vi "Build Json.vi"(8 "Error In":errorcluster, 11 "Asset":refnum<class "Asset.lvclass">) -> (0 "Error Out":errorcluster, 2 "JSON File Content":string, 3 "JSON File Name":string)   [LabVIEW 2019, in "Asset.lvclass"]
uses:
  Asset.lvclass
  AssetsJson.ctl
  AssetJson.ctl
  AssetLocationJson.ctl
  AssetExternalCalibrationJson.ctl
  ExternalCalibrationOperatorJson.ctl
  Asset Location/Asset Location.lvclass
  Asset External Calibration/Asset External Calibration.lvclass
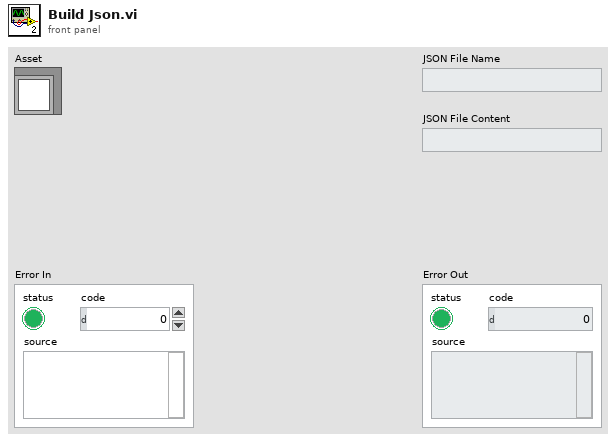
[diagram p1: front panel]
types:
  T1 = typedef "Asset.lvclass/AssetJson.ctl" = cluster{"serialNumber":string, "modelName":string, "modelNumber":u32, "vendorName":string, "vendorNumber":u32, "busType":string, "assetClass":string, "assetName":string, "firmwareVersion":string, "hardwareVersion":string, "location":T2, "supportsExternalCalibration":bool, "externalCalibration":T3, "name":string}
  T2 = typedef "Asset.lvclass/AssetLocationJson.ctl" = cluster{"slotNumber":u32, "parent":string}
  T3 = typedef "Asset.lvclass/AssetExternalCalibrationJson.ctl" = cluster{"date":string, "comments":string, "recommendedInterval":u32, "operator":T4, "temperatureSensors":cluster{"name":string, "reading":dbl}[], "nextRecommendedDate":string}
  T4 = typedef "Asset.lvclass/ExternalCalibrationOperatorJson.ctl" = cluster{"displayName":string, "userId":string}
  T5 = typedef "Asset.lvclass/AssetsJson.ctl" = cluster{"assets":T1[]}
  T6 = typedef "LVDateTimeRec.ctl" = cluster{"fractional second":dbl, "second":i32, "minute":i32, "hour":i32, "day of month":i32, "month":i32, "year":i32, "day of week":i32, "day of year":i32, "DST":i32}
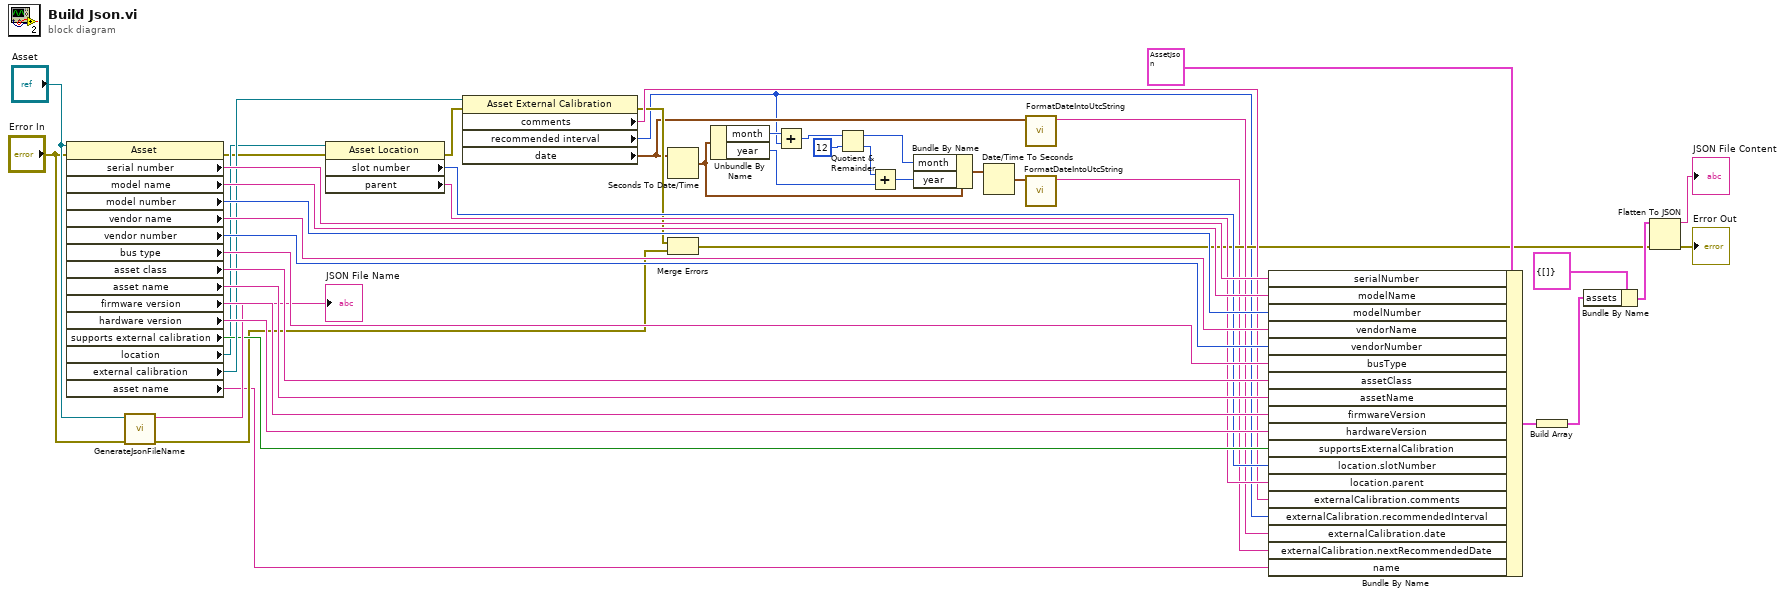
[diagram p0: block diagram]
diagram:
  n1 = property class="Asset"(reference="Asset", error in="Error In") -> (error out=w25:errorcluster, "serial number"=w46:string, "model name"=w45:string, "model number"=w44:u32, "vendor name"=w43:string, "vendor number"=w42:u32, "bus type"=w41:string, "asset class"=w40:string, "asset name"=w39:string, "firmware version"=w38:string, "hardware version"=w37:string, "supports external calibration"=w31:bool, "location"=w30:refnum<class "Asset Location.lvclass">, "external calibration"=w36:refnum<class "Asset External Calibration.lvclass">, "asset name"=w1:string)  [unwired: 1 out]
  n2 = call "GenerateJsonFileName.vi"("Error In"="Error In", "Asset"="Asset") -> ("Error Out"=w23:errorcluster, "File Name"=→"JSON File Name":string)  [unwired: 8 in]
  n3 = property class="Asset Location"(reference=w30, error in=w25) -> (error out=w19:errorcluster, "slot number"=w29:u32, "parent"=w28:string)  [unwired: 1 out]
  n4 = property class="Asset External Calibration"(reference=w36, error in=w19) -> (error out=w24:errorcluster, "comments"=w27:string, "recommended interval"=w10:u32, "date"=w13:timestamp)  [unwired: 1 out]
  n5 = Seconds To Date/Time(time stamp (now)=w13) -> (date time rec=w12:T6)  [unwired: 1 in]
  n6 = Merge Errors(w24, w23) -> (w18:errorcluster)
  n7 = Unbundle By Name(w12) -> ("month"=w11:i32, "year"=w6:i32)
  n8 = Add(x=w11, y=w10) -> (x+y=w9:u32)
  n9 = Quotient & Remainder(x=w9, y=u32 12) -> (x-y*floor(x/y)=w7:u32, floor(x/y)=w5:u32)
  n10 = Add(x=w5, y=w6) -> (x+y=w4:u32)
  n11 = Bundle By Name(cluster=w12, "month"=w7, "year"=w4) -> (w3:T6)
  n12 = Date/Time To Seconds(2:w3) -> (0:w2:timestamp)  [unwired: 1 in]
  n13 = call "FormatDateIntoUtcString.vi"("Date (UTC)"=w13) -> ("Formatted Date (UTC)"=w26:string)  [unwired: 10 in]
  n14 = call "FormatDateIntoUtcString.vi"("Date (UTC)"=w2) -> ("Formatted Date (UTC)"=w14:string)  [unwired: 10 in]
  n15 = Bundle By Name(cluster=T1 {"serialNumber"="", "modelName"="", "modelNumber"=0, "vendorName"="", "vendorNumber"=0, "busType"="", "assetClass"="", "assetName"="", "firmwareVersion"="", "hardwareVersion"="", "location"={"slotNumber"=0, "parent"=""}, "supportsExternalCalibration"=FALSE, "externalCalibration"={"date"="", "comments"="", "recommendedInterval"=0, "operator"={"displayName"="", "userId"=""}, "temperatureSensors"=[], "nextRecommendedDate"=""}, "name"=""} ("Asset 2"), "serialNumber"=w46, "modelName"=w45, "modelNumber"=w44, "vendorName"=w43, "vendorNumber"=w42, "busType"=w41, "assetClass"=w40, "assetName"=w39, "firmwareVersion"=w38, "hardwareVersion"=w37, "supportsExternalCalibration"=w31, "location.slotNumber"=w29, "location.parent"=w28, "externalCalibration.comments"=w27, "externalCalibration.recommendedInterval"=w10, "externalCalibration.date"=w26, "externalCalibration.nextRecommendedDate"=w14, "name"=w1) -> (w16:T1)
  n16 = Build Array(w16) -> (w15:T1[])
  n17 = Bundle By Name(cluster=T5 {"assets"=[]} ("json"), "assets"=w15) -> (w20:T5)
  n18 = Flatten To JSON(anything=w20, error in (no error)=w18) -> (JSON string=→"JSON File Content":string, 11:→"Error Out":errorcluster)  [unwired: 1 in]
